vi "Configure Plant Displays.vi"(5 "Feedback Chart":refnum<vi>, 7 "Displacement Display":refnum<vi>, 8 "error in":errorcluster, 9 "Flow Display":refnum<vi>, 10 "Pressure Display":refnum<vi>, 11 "Sequence Executor in":refnum<class "Sequence Executor.lvclass">) -> (0 "error out":errorcluster, 3 "Sequence Executor out":refnum<class "Sequence Executor.lvclass">)   [LabVIEW 2026, in "Sequence Executor.lvclass"]
doc: "Stores the Pressure, Flow and Displacement numeric display references and the Feedback Chart reference. Companion of Configure.vi. Call it before Launch Root Actor. Null references are allowed."
uses:
  Sequence Executor.lvclass
  Sequence Executor.lvclass/Sequence Executor.ctl
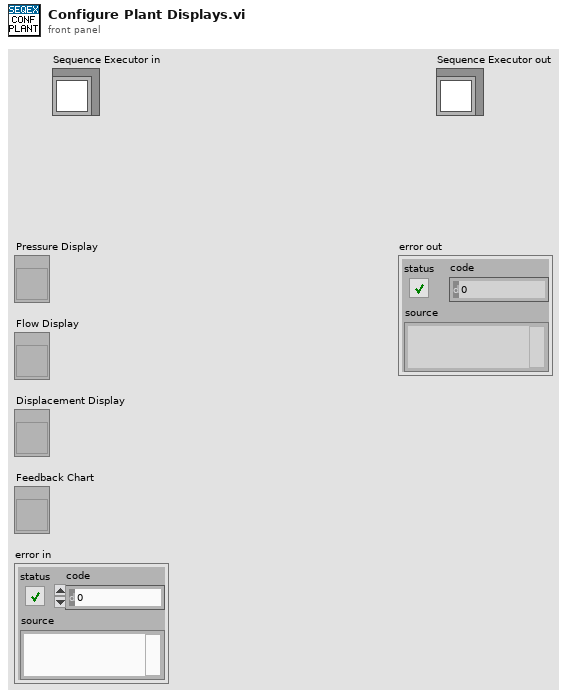
[diagram p1: front panel]
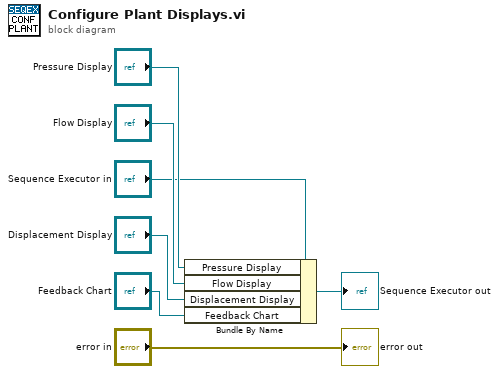
[diagram p0: block diagram]
diagram:
  n1 = Bundle By Name(cluster="Sequence Executor in", "Pressure Display"="Pressure Display", "Flow Display"="Flow Display", "Displacement Display"="Displacement Display", "Feedback Chart"="Feedback Chart") -> (→"Sequence Executor out":refnum<class "Sequence Executor.lvclass">)
  "error out" <- "error in"
